vi "Main.vi"() -> ()   [LabVIEW 2026]
doc: "This template is for the Queued Message Handler design pattern.\n\nThe Event Handling Loop generates messages based on user interface actions.\n\nThe Message Handling Loop processes messages generated by the Event Handling Loop, or by other messages. The messages are string values, so new messages can be added easily to the Message Cases case structure in the Message Handling Loop. Each message cluster can also provide an optional value for Message Data, which is a variant that can be converted to whatever message-specific data is required."
uses:
  controls/UI Data.ctl
  support/Message Queue/Enqueue Message (Single).vi
  <vilib>/Utility/error.llb/Error Cluster From Error Code.vi
  <vilib>/ErrorRing/Error Ring.xnode
  support/Message Queue/Message Queue.lvlib
  support/User Event - Stop/User Event - Stop.lvlib
panel:
  out "Waveform Graph":dbl[](graph)
  in  "Connect":bool
  in  "Exit":bool
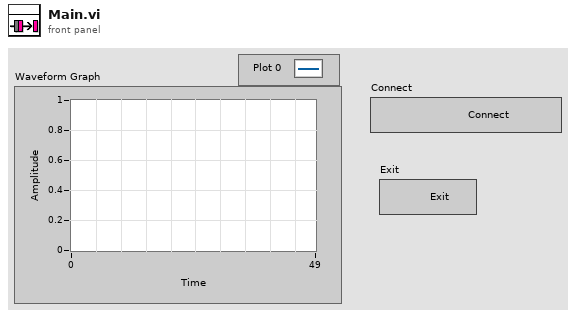
[diagram p1: front panel]
types:
  T1 = typedef "UI Data.ctl" = cluster{"connection ID":refnum<k5>, "Exit Button Ref":refnum<vi>}
  T2 = typedef "Message Queue.lvlib/All Message Queues.ctl" = cluster{"UI":refnum<queue>}
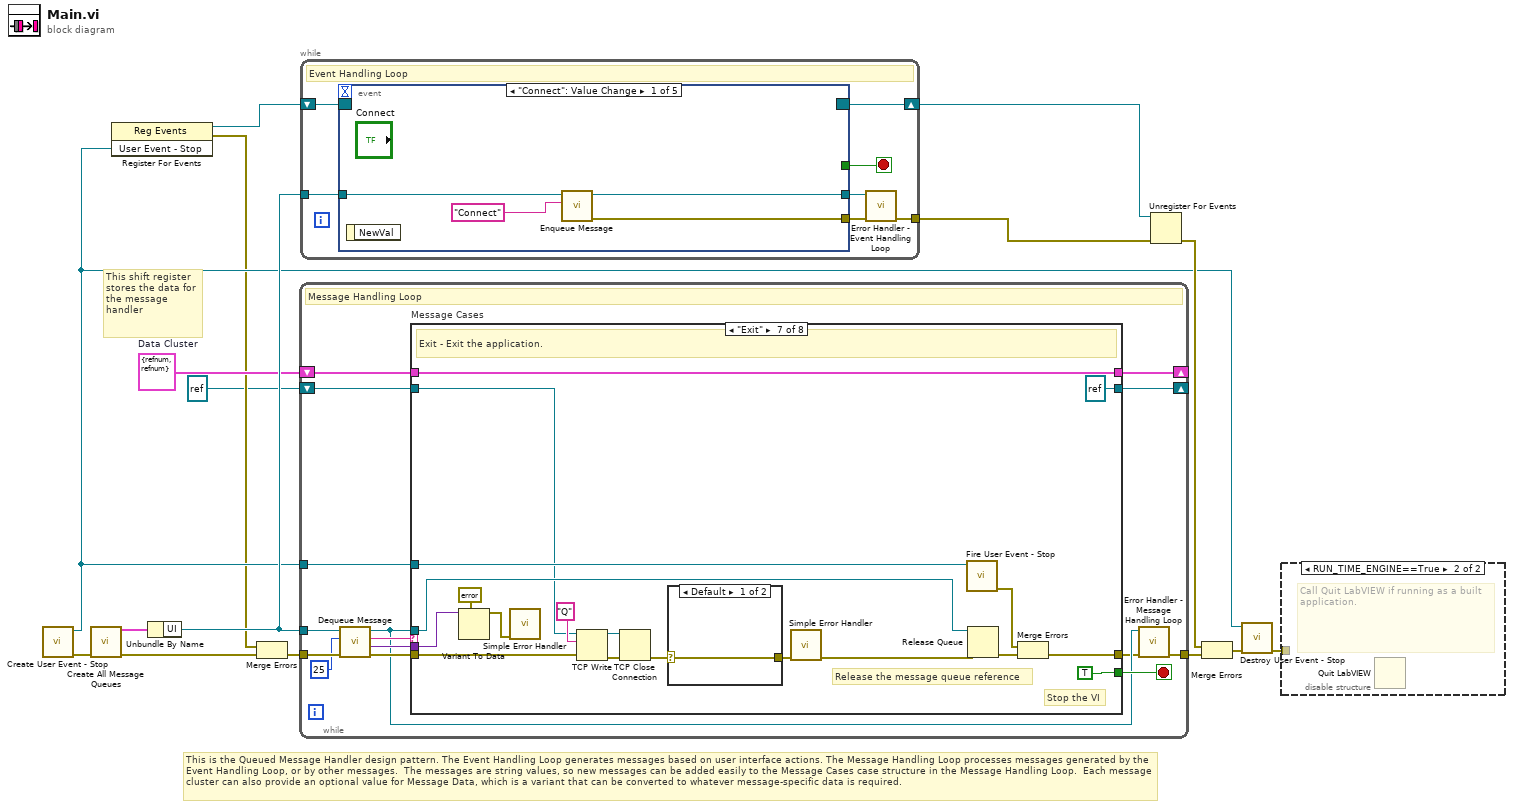
[diagram p0: block diagram]
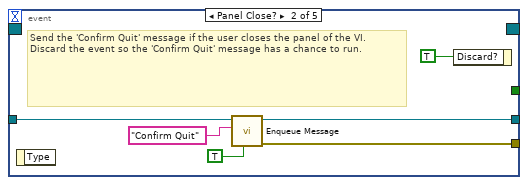
[diagram p3: hidden frame]
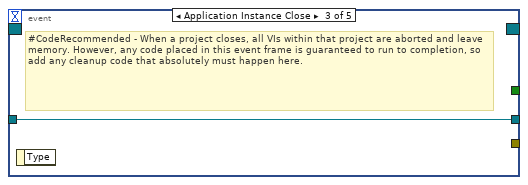
[diagram p4: hidden frame]
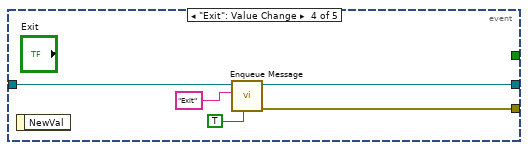
[diagram p5: hidden frame]
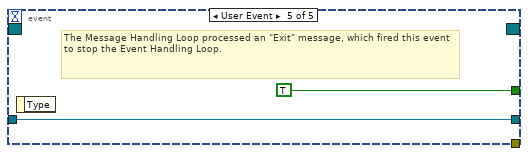
[diagram p6: hidden frame]
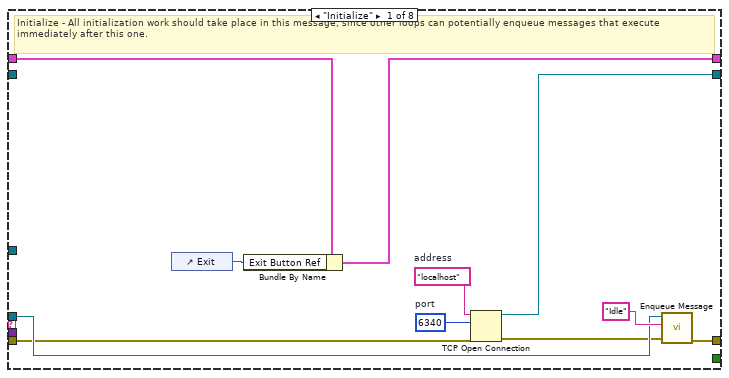
[diagram p7: hidden frame]
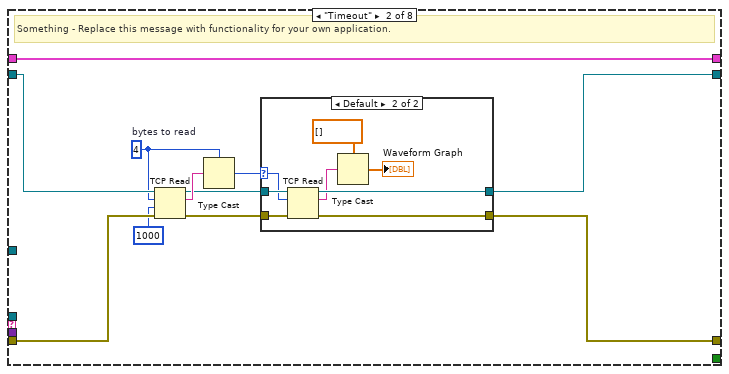
[diagram p8: hidden frame]
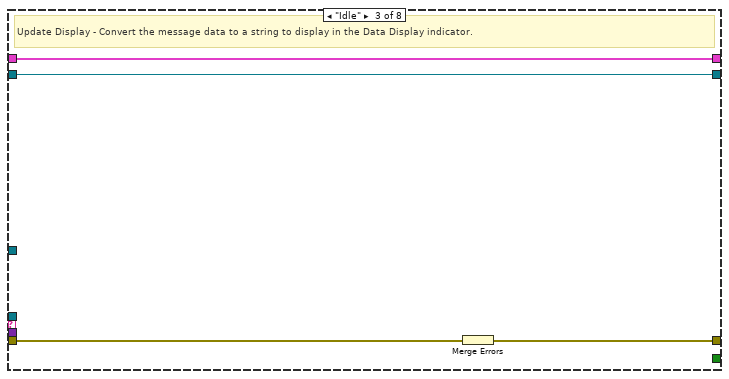
[diagram p10: hidden frame]
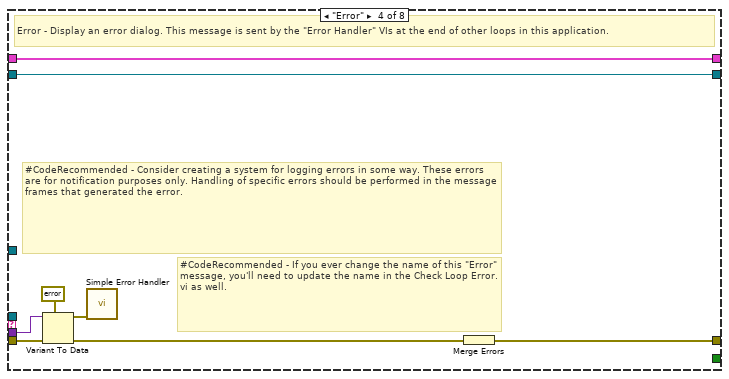
[diagram p11: hidden frame]
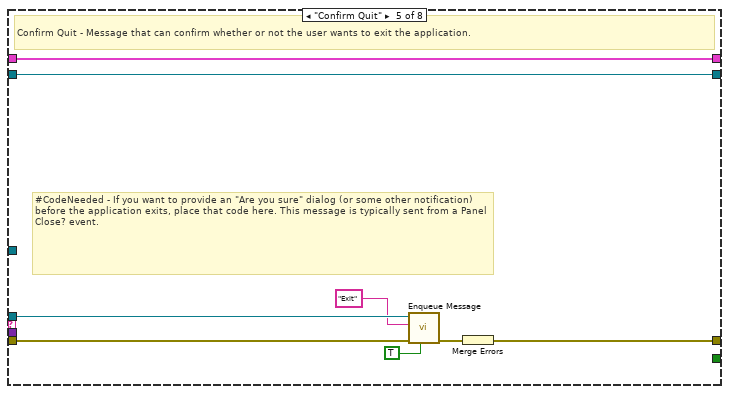
[diagram p12: hidden frame]
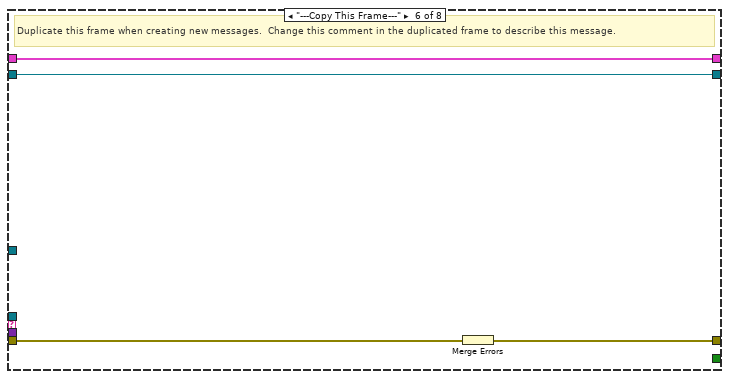
[diagram p13: hidden frame]
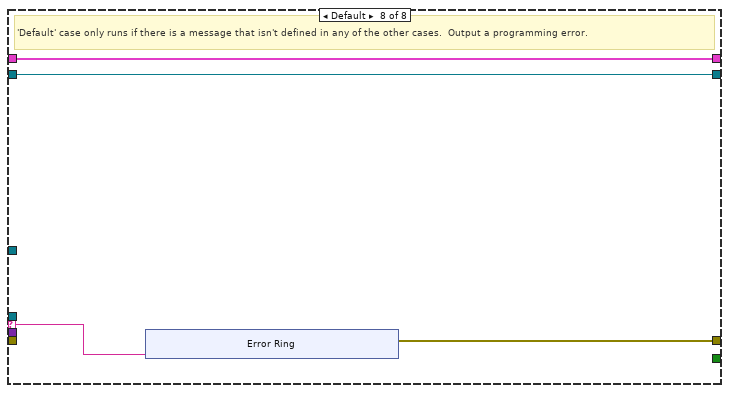
[diagram p15: hidden frame]
diagram:
  w8 = T1 {"connection ID"=refnum, "Exit Button Ref"=refnum}  # Data Cluster
  # "This is the Queued Message Handler design pattern. The Event Handling Loop generates messages based on user interface actions. The Message Handling Loop processes messages generated by the Event Handling Loop, or by other messages.  The messages are string values, so new messages can be added easily to the Message Cases case structure in the Message Handling Loop.  Each message cluster can also provide an optional value for Message Data, which is a variant that can be converted to whatever message-specific data is required."
  # "This shift register stores the data for the message handler"
  n1 = call "Create User Event - Stop.vi"() -> ("error out"=w12:errorcluster, "User Event - Stop"=w4:refnum<user-event>)  [unwired: 10 in]
  n2 = call "Create All Message Queues.vi"("error in (no error)"=w12) -> ("error out"=w16:errorcluster, "Message Queues out"=w15:T2)  [unwired: 9 in]
  n3 = register-events(w4) -> (reference out=w5:refnum<event-registration>, error out=w2:errorcluster)  [unwired: 2 in]
  n4 = Unbundle By Name(w15) -> ("UI"=w13:refnum<queue>)
  n5 = Merge Errors(w2, w16) -> (w3:errorcluster)
  n6 = while {
    tunnel: w13 -> [w23]
    shift-right: [w30] -> _
    shift-left: w8 -> [w31]
    tunnel: w4 -> [w28]
    tunnel: w3 -> [w27]
    tunnel: [w21] -> w14
    shift-right: [w19] -> _
    shift-left: refnum<k5> refnum ("connection ID") -> [w18]
    stop <- w29 stop-if-true
    # "Message Handling Loop"
    n7 = call "Dequeue Message.vi"("error in (no error)"=w27, "timeout in ms (-1)"=25, "Message Queue"=w23) -> ("error out"=w26:errorcluster, "Message Data"=w24:variant, "Message"=w25:string, "dup Message Queue"=w22:refnum<queue>)  [unwired: 5 in]
    n8 = case "Message Cases" shown="\"Exit\"" w25 {
      selector: w25 -> [_ _ _ _ _ _ _ w110]
      tunnel: w22 -> [w37 _ _ _ w79 _ w90 _]
      tunnel: w26 -> [w34 w52 w64 w75 w83 w87 w92 _]
      tunnel: [w42 w49 w66 w69 w81 w85 w103 w111] -> w20
      tunnel: w31 -> [w41 w53 w67 w74 w82 w86 w106 w112]
      tunnel: [w40 w53 w67 w74 w82 w86 w106 w112] -> w30
      tunnel: [_ _ _ _ _ _ TRUE _] -> w29
      tunnel: w24 -> [_ _ _ w73 _ _ w98 _]
      tunnel: w28 -> [_ _ _ _ _ _ w102 _]
      tunnel: [w32 w50 w65 w68 w76 w84 refnum<k5> refnum ("connection ID") w109] -> w19
      tunnel: w18 -> [_ w51 w65 w68 w76 w84 w89 w109]
      frame "Initialize" {
        w36 = u16 6340  # port
        w35 = "localhost"  # address
        # "Initialize - All initialization work should take place in this message, since other loops can potentially enqueue messages that execute immediately after this one."
        n9 = control-ref of="Exit"() -> (w39:refnum<vi>)
        n10 = Bundle By Name(cluster=w41, "Exit Button Ref"=w39) -> (w40:T1)
        n11 = TCP Open Connection(address=w35, remote port or service name=w36, error in (no error)=w34) -> (connection ID=w32:refnum<k5>, error out=w33:errorcluster)  [unwired: 2 in]
        n12 = call-poly "Enqueue Message.vi"("error in (no error)"=w33, "Message"="Idle", "Message Queue"=w37) -> ("error out"=w42:errorcluster)  [unwired: 7 in, 1 out]
      }
      frame "Timeout" {
        w45 = 4  # bytes to read
        # "Something - Replace this message with functionality for your own application."
        n13 = TCP Read(connection ID=w51, bytes to read=w45, error in (no error)=w52, 9:1000 ("timeout ms (25000)")) -> (connection ID out=w47:refnum<k5>, data out=w48:string, error out=w46:errorcluster)  [unwired: 1 in]
        n14 = Type Cast(type=w45, x=w48) -> (*(type *) &x=w44:i32)
        n15 = case shown="Default" w44 {
          selector: w44 -> [_ w56]
          tunnel: w47 -> [w55 w63]
          tunnel: w46 -> [w54 w62]
          tunnel: [w55 w59] -> w50
          tunnel: [w54 w58] -> w49
          frame ..0 {
            # "The server has not written any data"
          }
          frame Default {
            n16 = TCP Read(connection ID=w63, bytes to read=w56, error in (no error)=w62) -> (connection ID out=w59:refnum<k5>, data out=w57:string, error out=w58:errorcluster)  [unwired: 2 in]
            n17 = Type Cast(type=dbl[] [] ("chart"), x=w57) -> (*(type *) &x=→"Waveform Graph":dbl[])
          }
        }
      }
      frame "Idle" {
        # "Update Display - Convert the message data to a string to display in the Data Display indicator."
        n18 = Merge Errors(w64) -> (w66:errorcluster)
      }
      frame "Error" {
        # "#CodeRecommended - If you ever change the name of this \"Error\" message, you'll need to update the name in the Check Loop Error.vi as well."
        # "#CodeRecommended - Consider creating a system for logging errors in some way. These errors are for notification purposes only. Handling of specific errors should be performed in the message frames that generated the error."
        # "Error - Display an error dialog. This message is sent by the \"Error Handler\" VIs at the end of other loops in this application."
        n19 = Variant To Data(error in=w75, type=errorcluster {"status"=FALSE, "code"=0, "source"=""} ("error constant"), Variant=w73) -> (data=w71:errorcluster, error out=w70:errorcluster)
        n20 = call <vilib>:"Simple Error Handler.vi"("error in (no error)"=w71) -> ()  [unwired: 4 in, 5 out]
        n21 = Merge Errors(w70) -> (w69:errorcluster)
      }
      frame "Confirm Quit" {
        # "#CodeNeeded - If you want to provide an \"Are you sure\" dialog (or some other notification) before the application exits, place that code here. This message is typically sent from a Panel Close? event."
        # "Confirm Quit - Message that can confirm whether or not the user wants to exit the application."
        n22 = call-poly "Enqueue Message.vi"("Priority Message? (F)"=TRUE, "error in (no error)"=w83, "Message"="Exit", "Message Queue"=w79) -> ("error out"=w80:errorcluster)  [unwired: 6 in, 1 out]
        n23 = Merge Errors(w80) -> (w81:errorcluster)
      }
      frame "---Copy This Frame---" {
        # "Duplicate this frame when creating new messages.  Change this comment in the duplicated frame to describe this message."
        n24 = Merge Errors(w87) -> (w85:errorcluster)
      }
      frame "Exit" {
        # "Stop the VI"
        # "Release the message queue reference"
        # "Exit - Exit the application."
        n25 = Variant To Data(type=errorcluster {"status"=FALSE, "code"=0, "source"=""} ("error constant"), Variant=w98) -> (data=w99:errorcluster)  [unwired: 1 in, 1 out]
        n26 = call <vilib>:"Simple Error Handler.vi"("error in (no error)"=w99) -> ()  [unwired: 4 in, 5 out]
        n27 = TCP Write(connection ID=w89, data in="Q", error in (no error)=w92) -> (connection ID out=w97:refnum<k5>, error out=w96:errorcluster)  [unwired: 2 out]
        n28 = TCP Close Connection(connection ID=w97, error in (no error)=w96) -> (error out=w94:errorcluster)  [unwired: 1 in, 1 out]
        n29 = case shown="Default" w94 {
          selector: w94 -> [w107 w108]
          tunnel: [w107 w108] -> w93
          frame #0 {
          }
          frame #1 {
          }
        }
        n30 = call <vilib>:"Simple Error Handler.vi"("error in (no error)"=w93) -> ("error out"=w91:errorcluster)  [unwired: 4 in, 4 out]
        n31 = call "Fire User Event - Stop.vi"("User Event - Stop"=w102) -> ("error out"=w101:errorcluster)  [unwired: 10 in]
        n32 = Release Queue(queue=w90, error in (no error)=w91) -> (error out=w104:errorcluster)  [unwired: 1 in, 2 out]
        n33 = Merge Errors(w101, w104) -> (w103:errorcluster)
      }
      frame Default {
        # "'Default' case only runs if there is a message that isn't defined in any of the other cases.  Output a programming error."
        n34 = xnode "Error Ring"("parameter 0"=w110) -> ("error out"=w111:errorcluster)
      }
    }
    n35 = call "Error Handler - Message Handling Loop.vi"("error in (no error)"=w20, "Message Queue"=w22) -> ("dup error in"=w21:errorcluster)  [unwired: 8 in, 1 out]
  }
  n36 = while {
    tunnel: w13 -> [w126]
    shift-right: [w124] -> w9
    shift-left: w5 -> [w125]
    tunnel: [w120] -> w6
    stop <- w122 stop-if-true
    # "Event Handling Loop"
    n37 = event shown="[0] \"Connect\": Value Change" {
      selector: w125 -> [_ _ _ _ _]
      dyn-events: [_ _ _ _ _] -> w124
      timeout: _ -> [_ _ _ _ _]
      tunnel: [_ _ _ _ TRUE ("Discard?")] -> w122
      tunnel: w126 -> [w130 w135 w137 w142 w144]
      tunnel: [w127 w134 _ w141 _] -> w123
      tunnel: [w129 w133 w137 w140 w144] -> w121
      event "Connect": Value Change {
        n38 = event-data() -> ()  [unwired: 1 in, 1 out]
        n39 = call-poly "Enqueue Message.vi"("Message"="Connect", "Message Queue"=w130) -> ("error out"=w127:errorcluster, "dup Message Queue"=w129:refnum<queue>)  [unwired: 8 in]
      }
      event Panel Close? {
        # "Send the 'Confirm Quit' message if the user closes the panel of the VI. Discard the event so the 'Confirm Quit' message has a chance to run."
        n40 = event-data() -> ()  [unwired: 1 in, 1 out]
        n41 = call-poly "Enqueue Message.vi"("Priority Message? (F)"=TRUE, "Message"="Confirm Quit", "Message Queue"=w135) -> ("error out"=w134:errorcluster, "dup Message Queue"=w133:refnum<queue>)  [unwired: 7 in]
        n42 = event-data("Discard?"=TRUE) -> ()  [unwired: 1 in, 1 out]
      }
      event Application Instance Close {
        # "#CodeRecommended - When a project closes, all VIs within that project are aborted and leave memory. However, any code placed in this event frame is guaranteed to run to completion, so add any cleanup code that absolutely must happen here."
        n43 = event-data() -> ()  [unwired: 1 in, 1 out]
      }
      event "Exit": Value Change {
        n44 = event-data() -> ()  [unwired: 1 in, 1 out]
        n45 = call-poly "Enqueue Message.vi"("Priority Message? (F)"=TRUE, "Message"="Exit", "Message Queue"=w142) -> ("error out"=w141:errorcluster, "dup Message Queue"=w140:refnum<queue>)  [unwired: 7 in]
      }
      event User Event {
        # "The Message Handling Loop processed an \"Exit\" message, which fired this event to stop the Event Handling Loop."
        n46 = event-data() -> ()  [unwired: 1 in, 1 out]
      }
    }
    n47 = call "Error Handler - Event Handling Loop.vi"("error in (no error)"=w123, "Message Queue"=w121) -> ("dup error in"=w120:errorcluster)  [unwired: 8 in, 1 out]
  }
  n48 = Unregister For Events(event registration refnum=w9, error in=w6) -> (error out=w10:errorcluster)
  n49 = Merge Errors(w10, w14) -> (w11:errorcluster)
  n50 = call "Destroy User Event - Stop.vi"("error in (no error)"=w11, "User Event - Stop"=w4) -> ("error out"=w7:errorcluster)  [unwired: 9 in]
  n51 = disable-structure shown="RUN_TIME_ENGINE==True" {
    disable-tunnel: w7 -> [_ _]
    frame condition #0 (active) {
    }
    frame condition #1 {
      # "Call Quit LabVIEW if running as a built application."
      n52 = Quit LabVIEW() -> ()  [unwired: 1 in]
    }
  }
